vi "Teleop.vi"(10 "Match Info":T1={"Autonomous Elapsed Seconds"=0.0, "TeleOp Elapsed Seconds"=0.0, "Disabled Elapsed Seconds"=0.0, "Visited Autonomous"=FALSE, "Visited TeleOp"=FALSE, "Visited Disabled"=FALSE, "Autonomous Settings"={"Autonomous Style"=enum."Independent", "VI Refnum"=refnum}}, 11 "Call Context":T2) -> ()   [LabVIEW 2020]
doc: "This VI is called for each TeleOp packet received from the DS where the robot is not disabled. It is often used to read from the joysticks and update I/O or to update setpoints for timed control loops. It should complete and return within 20 milliseconds or it may miss DS packets."
uses:
  <vilib>/Rock Robotics/WPI/DriverStation/WPI_DriverStationDerivedRobotMode.ctl
  <vilib>/Rock Robotics/WPI/DriverStation/WPI_DriverStationMatch Info.ctl
  <vilib>/Rock Robotics/WPI/Solenoid/WPI_SolenoidValue.ctl
  <vilib>/Rock Robotics/WPI/Utilities/WPI_GetSetVariantRefNum.vi
  <vilib>/Rock Robotics/WPI/Solenoid/Deprecated/WPI_SolenoidSetBool.vi
  <vilib>/Rock Robotics/Network Tables/NT Write Number.vi
  <vilib>/Rock Robotics/WPI/Solenoid/WPI_SolenoidSetEnum.vi
  Robot Global Data.vi
panel:
  # "April tags"
  # "Retroreflective tape"
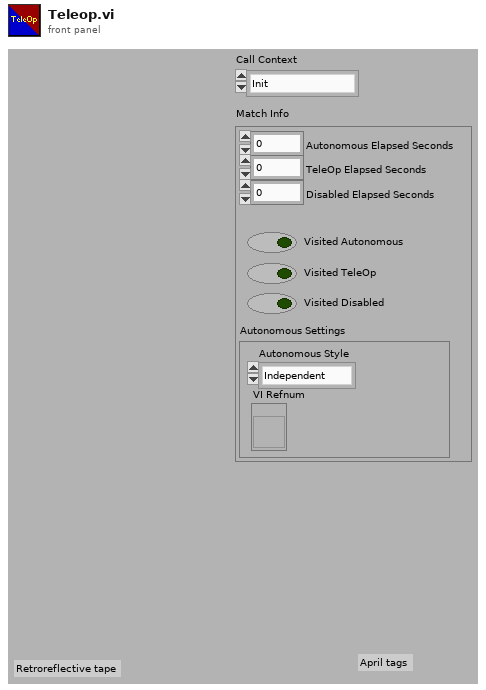
[diagram p1: front panel]
types:
  T1 = typedef "WPI_DriverStationMatch Info.ctl" = cluster{"Autonomous Elapsed Seconds":dbl, "TeleOp Elapsed Seconds":dbl, "Disabled Elapsed Seconds":dbl, "Visited Autonomous":bool, "Visited TeleOp":bool, "Visited Disabled":bool, "Autonomous Settings":cluster{"Autonomous Style":enum16{"Iterative", "Independent"}, "VI Refnum":refnum<vi>}}
  T2 = typedef "WPI_DriverStationDerivedRobotMode.ctl" = enum16{"Init", "Execute", "Stop"}
  T3 = typedef "WPI_SolenoidValue.ctl" = enum16{"Off", "On", "Forward", "Reverse"}
  T4 = typedef "WPI_JoystickDevRef.ctl" = cluster{"Device":T5}
  T5 = typedef "WPI_JoystickDeviceEnum.ctl" = enum16{"USB 0", "USB 1", "USB 2", "USB 3", "USB 4", "USB 5"}
  T6 = cluster{"Axes[0]":dbl, "Axes[1]":dbl, "Axes[2]":dbl, "Axes[3]":dbl, "Axes[4]":dbl, "Axes[5]":dbl, "Axes[6]":dbl, "Axes[7]":dbl, "Axes[8]":dbl}
  T7 = cluster{"Buttons[0]":bool, "Buttons[1]":bool, "Buttons[2]":bool, "Buttons[3]":bool, "Buttons[4]":bool, "Buttons[5]":bool, "Buttons[6]":bool, "Buttons[7]":bool, "Buttons[8]":bool}
  T8 = typedef "WPI_SolenoidDevRef.ctl" = cluster{"DevStatus":errorcluster, "Pneumatics Control Module":u8, "Forward Solenoid Channel":T9, "Reverse Solenoid Channel":T9}
  T9 = typedef "WPI_SolenoidChannel.ctl" = enum8{"Solenoid 0", "Solenoid 1", "Solenoid 2", "Solenoid 3", "Solenoid 4", "Solenoid 5", "Solenoid 6", "Solenoid 7", "Solenoid 8", "Solenoid 9", "Solenoid 10", "Solenoid 11", "Solenoid 12", "Solenoid 13", "Solenoid 14", "Solenoid 15", "Invalid"}
  T10 = typedef "WPI_MotorControlDeviceRef.ctl" = cluster{"DeviceStatus":errorcluster, "Type":T11, "PWM":cluster{"PWM Channel":T12, "DeadBand":T13}, "CAN":cluster{"Device Number":u8, "SetOutput VI Ref":variant, "GetOutput VI Ref":variant, "Enable VI Ref":variant, "Disable VI Ref":variant, "Data":variant}, "Invert":bool, "DIO PWM":cluster{"PWM \"Enable\" Channel":T12, "DIOChannel":T14, "PWM Rate":dbl}}
  T11 = typedef "WPI_MotorControlType.ctl" = enum16{"PWM", "CAN", "DIO PWM"}
  T12 = typedef "FPGA_DIOPWMChannel.ctl" = enum8{"PWM 0", "PWM 1", "PWM 2", "PWM 3", "PWM 4", "PWM 5", "PWM 6", "PWM 7", "PWM 8", "PWM 9", "PWM MXP 0", "PWM MXP 1", "PWM MXP 2", "PWM MXP 3", "PWM MXP 4", "PWM MXP 5", "PWM MXP 6", "PWM MXP 7", "PWM MXP 8", "PWM MXP 9", "Invalid"}
  T13 = typedef "WPI_PWMDeadband.ctl" = cluster{"Name":string, "maxPositivePwm":i32, "minPositivePwm":i32, "centerPwm":i32, "maxNegativePwm":i32, "minNegativePwm":i32, "angularRange":u16}
  T14 = typedef "FPGA_DIOChannel.ctl" = enum8{"DIO 0", "DIO 1", "DIO 2", "DIO 3", "DIO 4", "DIO 5", "DIO 6", "DIO 7", "DIO 8", "DIO 9", "DIO MXP 0", "DIO MXP 1", "DIO MXP 2", "DIO MXP 3", "DIO MXP 4", "DIO MXP 5", "DIO MXP 6", "DIO MXP 7", "DIO MXP 8", "DIO MXP 9", "DIO MXP 10", "DIO MXP 11", "DIO MXP 12", "DIO MXP 13", "DIO MXP 14", "DIO MXP 15", "SPI Port CS1", "SPI Port CS2", "SPI Port CS3", "SPI Port MISO", "SPI Port MOSI", "Invalid"}
  T15 = typedef "WPI_RobotDriveDevRef.ctl" = cluster{"DevStatus":errorcluster, "Motors[]":T10[], "Square Inputs":bool, "Max Output":dbl}
  T16 = cluster{"Motors[][0]":T10, "Motors[][1]":T10, "Motors[][2]":T10, "Motors[][3]":T10, "Motors[][4]":T10, "Motors[][5]":T10, "Motors[][6]":T10, "Motors[][7]":T10, "Motors[][8]":T10}
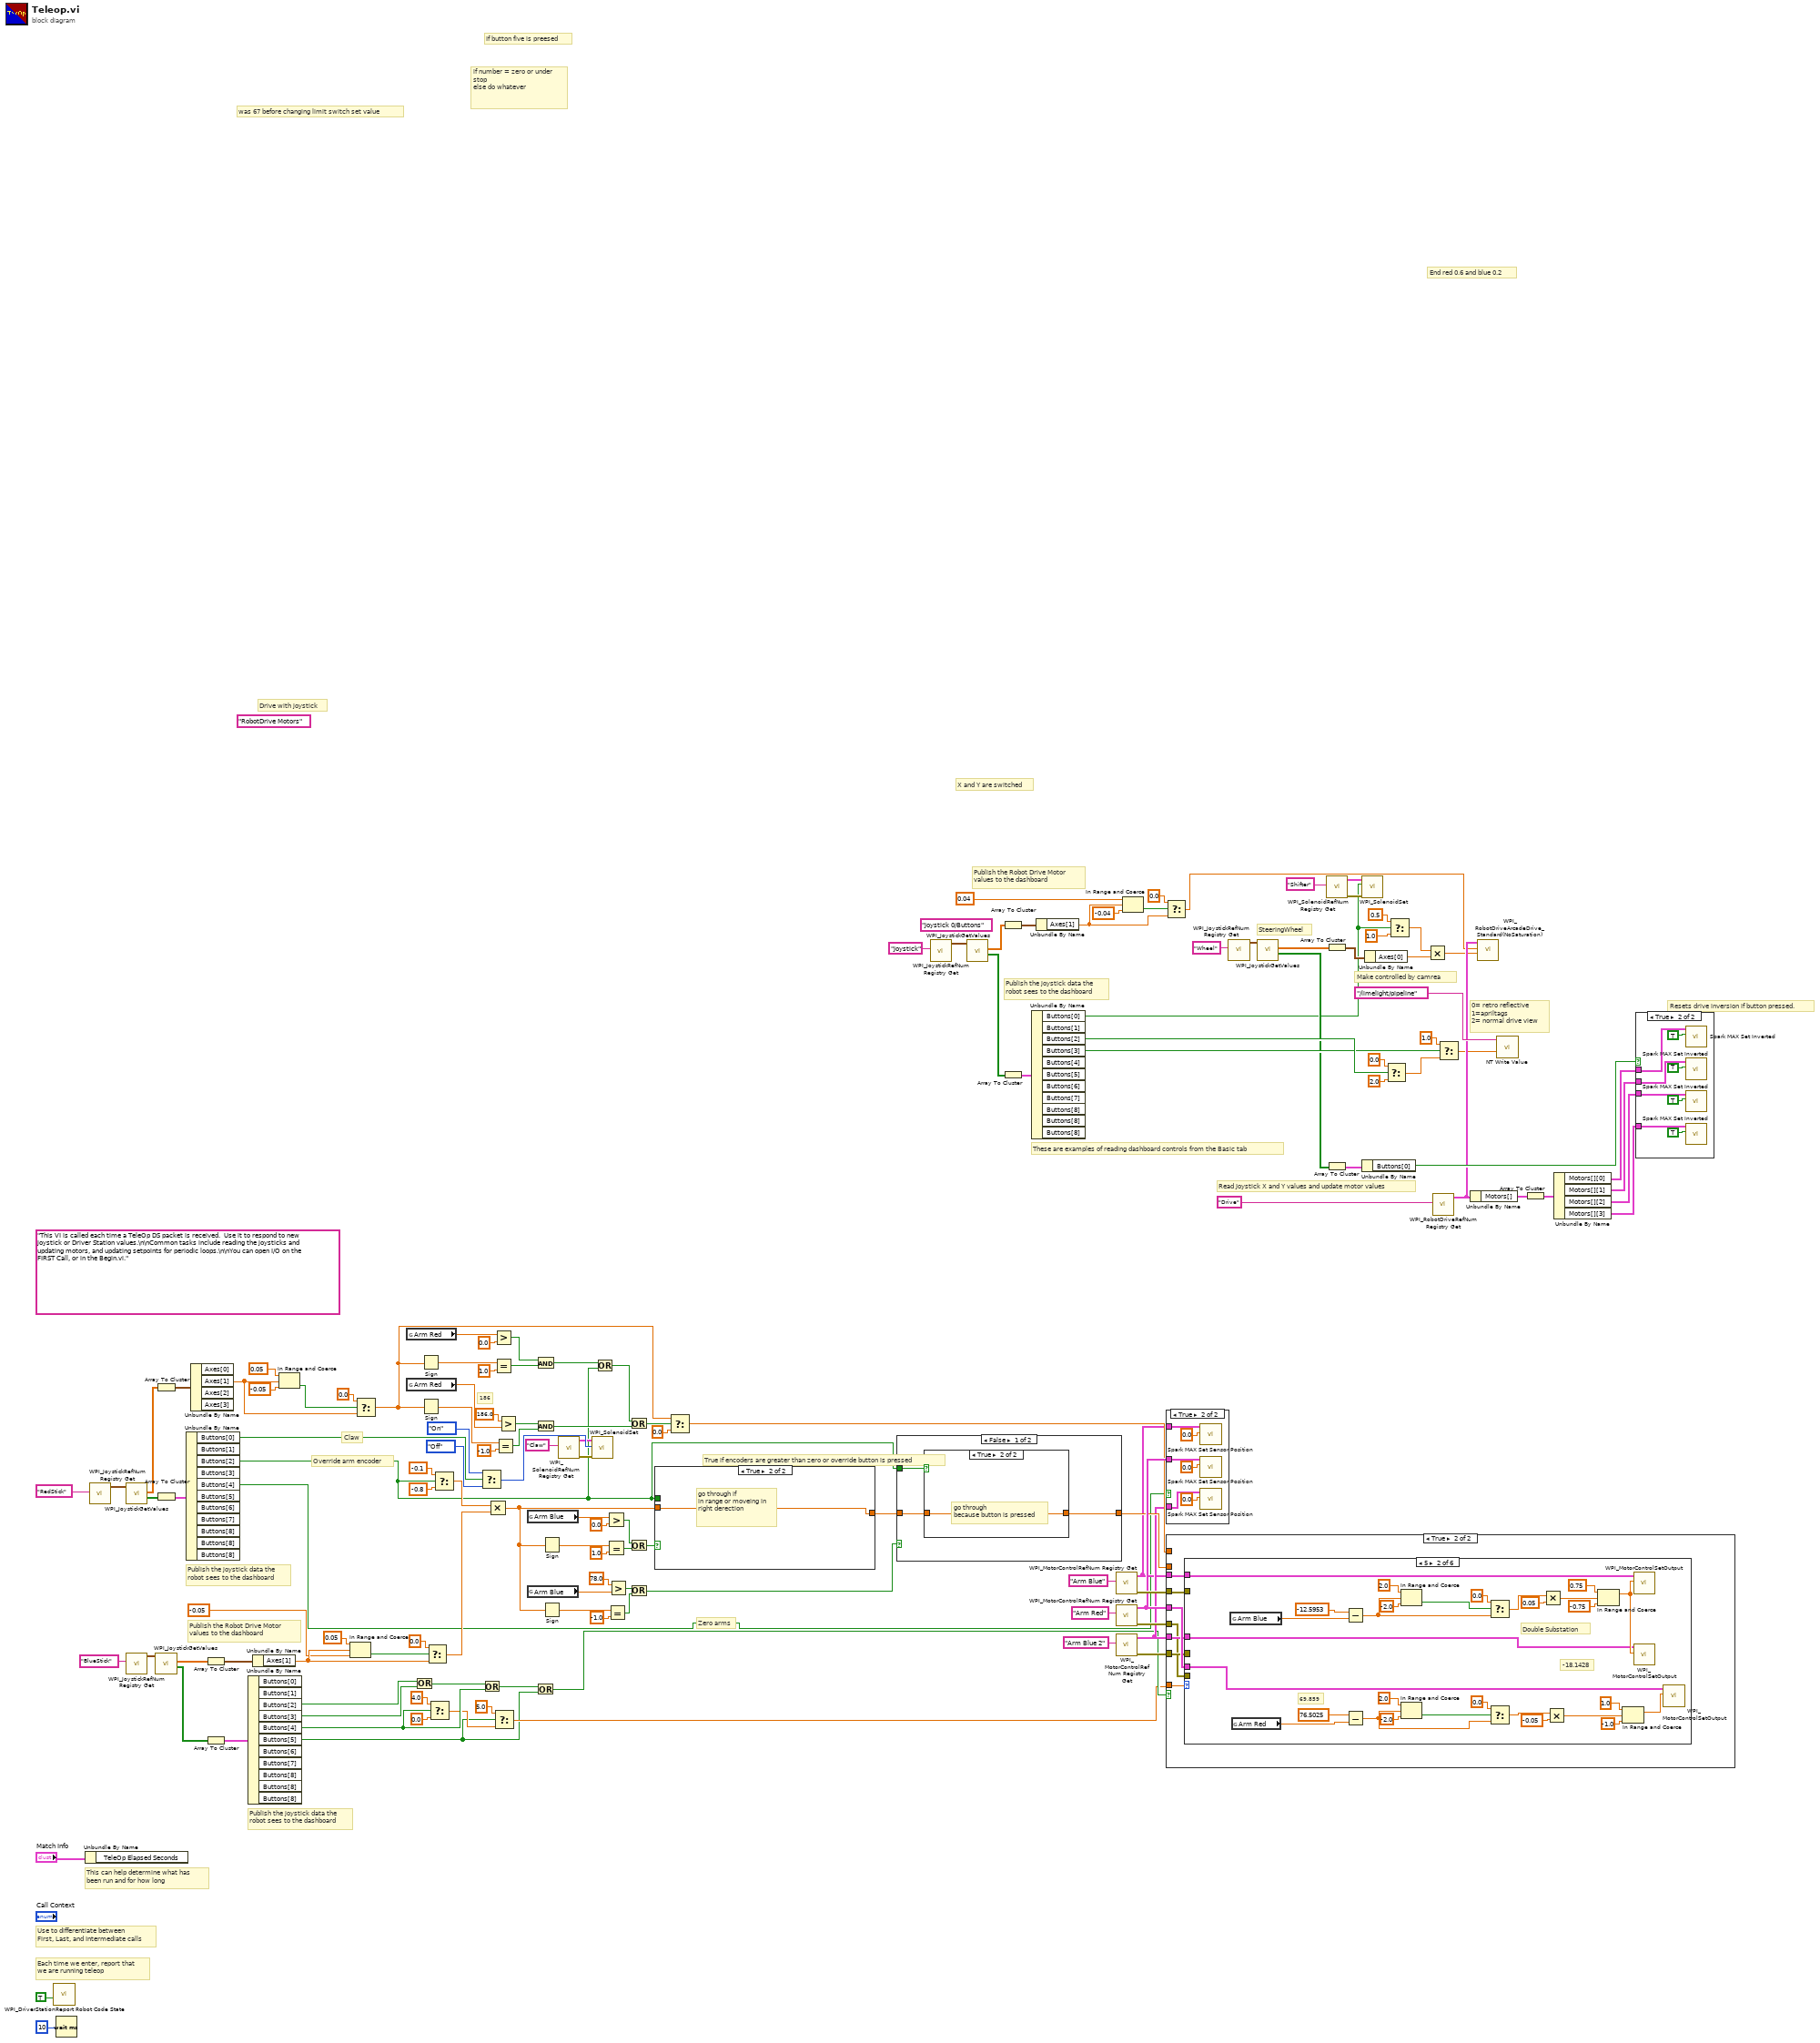
[diagram p0: block diagram]
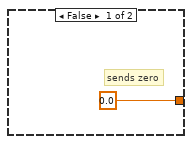
[diagram p2: hidden frame]
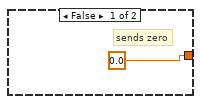
[diagram p5: hidden frame]
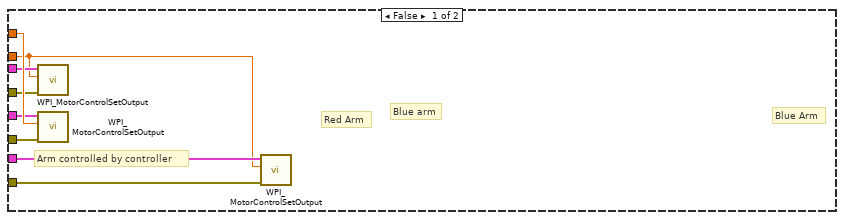
[diagram p8: hidden frame]
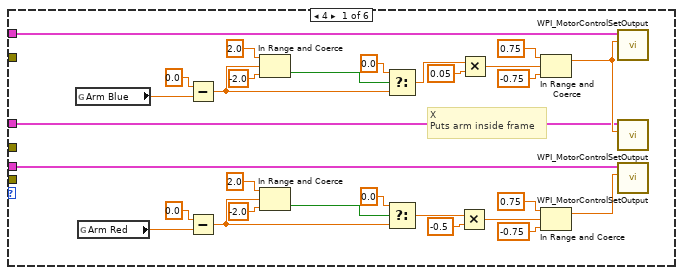
[diagram p9: hidden frame]
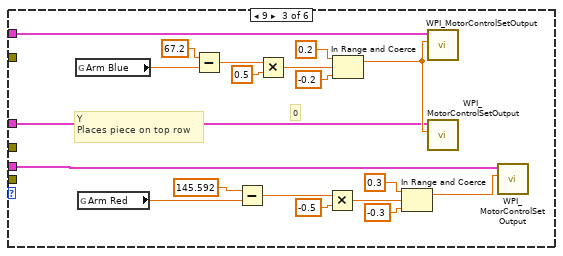
[diagram p10: hidden frame]
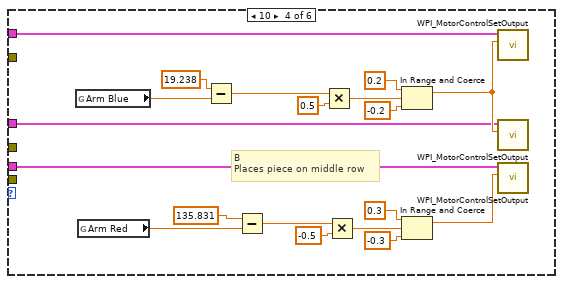
[diagram p11: hidden frame]
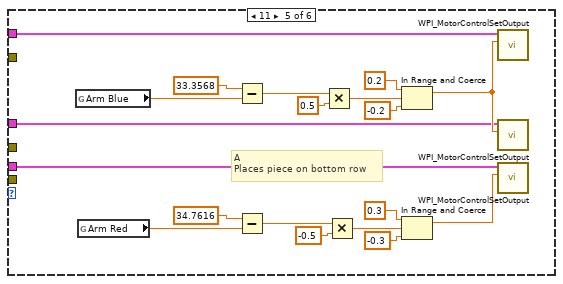
[diagram p12: hidden frame]
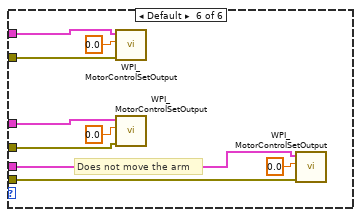
[diagram p13: hidden frame]
diagram:
  (unwired) "RobotDrive Motors" ("Name")
  (unwired) "Joystick 0/Buttons" ("Name")
  (unwired) "This VI is called each time a TeleOp DS packet is received.  Use it to respond to new joystick or Driver Station values.\n\nCommon tasks include reading the joysticks and updating motors, and updating setpoints for periodic loops.\n\nYou can open I/O on the FIRST Call, or in the Begin.vi."
  # "Drive with joystick"
  # "186"
  # "End red 0.6 and blue 0.2"
  # "Zero arms"
  # "Override arm encoder"
  # "Claw"
  # "Publish the Robot Drive Motor\nvalues to the dashboard"
  # "Publish the joystick data the\nrobot sees to the dashboard"
  # "Publish the joystick data the\nrobot sees to the dashboard"
  # "X and Y are switched"
  # "was 67 before changing limit switch set value"
  # "True if encoders are greater than zero or override button is pressed"
  # "if number = zero or under\nstop\nelse do whatever"
  # "If button five is preesed"
  # "Resets drive inversion if button pressed."
  # "0= retro reflective\n1=apriltags\n2= normal drive view"
  # "Make controlled by camrea"
  # "SteeringWheel"
  # "These are examples of reading dashboard controls from the Basic tab"
  # "Publish the Robot Drive Motor\nvalues to the dashboard"
  # "Publish the joystick data the\nrobot sees to the dashboard"
  # "Each time we enter, report that\nwe are running teleop"
  # "Use to differentiate between\nFirst, Last, and Intermediate calls"
  # "This can help determine what has\nbeen run and for how long"
  # "Read Joystick X and Y values and update motor values"
  n1 = call <vilib>:"WPI_DriverStationReport Robot Code State.vi"("TeleOp"=TRUE ("Autonomous")) -> ()  [unwired: 10 in, 1 out]
  n2 = Wait (ms)(milliseconds to wait=u32 10) -> ()  [unwired: 1 out]
  n3 = Unbundle By Name("Match Info") -> ()  [unwired: 1 out]
  n4 = call <vilib>:"WPI_JoystickRefNum Registry Get.vi"("refnum name"="RedStick") -> ("JoystickDevRef"=w39:T4)  [unwired: 1 in, 9 out]
  n5 = call <vilib>:"WPI_JoystickGetValues.vi"("JoystickDevRef"=w39) -> ("Buttons"=w36:bool[], "Axes"=w38:dbl[])  [unwired: 6 in, 3 out]
  n6 = call <vilib>:"WPI_JoystickRefNum Registry Get.vi"("refnum name"="BlueStick") -> ("JoystickDevRef"=w26:T4)  [unwired: 1 in, 9 out]
  n7 = Array To Cluster(array=w38) -> (cluster=w37:T6)
  n8 = Array To Cluster(array=w36) -> (cluster=w35:T7)
  n9 = call <vilib>:"WPI_JoystickGetValues.vi"("JoystickDevRef"=w26) -> ("Buttons"=w29:bool[], "Axes"=w27:dbl[])  [unwired: 6 in, 3 out]
  n10 = Unbundle By Name(w35) -> ("Buttons[0]"=w14:bool, "Buttons[2]"=w22:bool, "Buttons[4]"=w23:bool)  [unwired: 8 out]
  n11 = Unbundle By Name(w37) -> ("Axes[1]"=w18:dbl)  [unwired: 3 out]
  n12 = Array To Cluster(array=w27) -> (cluster=w28:T6)
  n13 = Array To Cluster(array=w29) -> (cluster=w30:T7)
  n14 = Unbundle By Name(w30) -> ("Buttons[2]"=w8:bool, "Buttons[3]"=w9:bool, "Buttons[4]"=w6:bool, "Buttons[5]"=w2:bool)  [unwired: 7 out]
  n15 = Unbundle By Name(w28) -> ("Axes[1]"=w34:dbl)
  n16 = In Range and Coerce(upper limit=0.05, x=w18, lower limit=-0.05) -> (In Range?=w19:bool)  [unwired: 1 out]
  n17 = In Range and Coerce(upper limit=0.05, x=w34, lower limit=-0.05) -> (In Range?=w31:bool)  [unwired: 1 out]
  n18 = Select(t=0.0, s=w19, f=w18) -> (s? t:f=w17:dbl)
  n19 = global read "Robot Global Data.vi" "Arm Red"() -> (w83:dbl)
  n20 = global read "Robot Global Data.vi" "Arm Red"() -> (w77:dbl)
  n21 = Or(x=w8, y=w9) -> (x .or. y?=w13:bool)
  n22 = Sign(1:w17) -> (0:w81:dbl)
  n23 = Sign(1:w17) -> (0:w79:dbl)
  n24 = Select(t=0.0, s=w31, f=w34) -> (s? t:f=w24:dbl)
  n25 = Select(t=4.0, s=w6, f=0.0) -> (s? t:f=w3:dbl)
  n26 = Select(t=-0.1, s=w22, f=-0.8) -> (s? t:f=w45:dbl)
  n27 = Select(t=WPI_SolenoidValue."On" ("Value"), s=w14, f=WPI_SolenoidValue."Off" ("Value")) -> (s? t:f=w62:T3)
  n28 = Or(x=w13, y=w6) -> (x .or. y?=w12:bool)
  n29 = Multiply(x=w45, y=w24) -> (x*y=w42:dbl)
  n30 = Greater?(x=w83, y=0.0) -> (0:w75:bool)
  n31 = Equal?(x=w81, y=1.0) -> (x = y?=w74:bool)
  n32 = Select(t=5.0, s=w2, f=w3) -> (s? t:f=w7:dbl)
  n33 = Equal?(x=w79, y=-1.0) -> (x = y?=w73:bool)
  n34 = Greater?(x=186.0 ("y"), y=w77) -> (0:w72:bool)
  n35 = global read "Robot Global Data.vi" "Arm Blue"() -> (w99:dbl)
  n36 = global read "Robot Global Data.vi" "Arm Blue"() -> (w87:dbl)
  n37 = Or(x=w12, y=w2) -> (x .or. y?=w11:bool)
  n38 = And(x=w75, y=w74) -> (x .and. y?=w71:bool)
  n39 = And(x=w72, y=w73) -> (x .and. y?=w70:bool)
  n40 = Sign(1:w42) -> (0:w96:dbl)
  n41 = Sign(1:w42) -> (0:w91:dbl)
  n42 = call <vilib>:"WPI_SolenoidRefNum Registry Get.vi"("refnum name"="Claw") -> ("error out"=w58:errorcluster, "SolenoidDevRef"=w59:T8)  [unwired: 9 in]
  n43 = call-poly <vilib>:"WPI_SolenoidSet.vi"("error in (no error)"=w58, "Value"=w62, "SolenoidDevRef"=w59) -> ()  [unwired: 7 in, 2 out]
  n44 = Or(x=w71, y=w22) -> (x .or. y?=w69:bool)
  n45 = Greater?(x=w99, y=0.0) -> (0:w98:bool)
  n46 = Equal?(x=w96, y=1.0) -> (x = y?=w94:bool)
  n47 = Equal?(x=w91, y=-1.0) -> (x = y?=w89:bool)
  n48 = Greater?(x=78.0 ("y"), y=w87) -> (0:w92:bool)
  n49 = Or(x=w69, y=w70) -> (x .or. y?=w68:bool)
  n50 = Or(x=w98, y=w94) -> (x .or. y?=w93:bool)
  n51 = Or(x=w92, y=w89) -> (x .or. y?=w88:bool)
  n52 = case shown="True" w93 {
    tunnel: w22 -> [w142 _]
    tunnel: [w141 w145] -> w85
    tunnel: w42 -> [w140 w145]
    frame False {
      n53 = case shown="True" w142 {
        tunnel: [0.0 w144] -> w141
        tunnel: w140 -> [_ w144]
        frame False {
          # "sends zero"
        }
        frame True {
          # "go through\nbecause button is pressed"
        }
      }
    }
    frame True {
      # "go through if\nin range or moveing in right derection"
    }
  }
  n54 = Select(t=w17, s=w68, f=0.0) -> (s? t:f=w66:dbl)
  n55 = case shown="False" w88 {
    tunnel: w22 -> [w148 _]
    tunnel: [w147 w151] -> w84
    tunnel: w85 -> [w146 w151]
    frame False {
      n56 = case shown="True" w148 {
        tunnel: [0.0 w150] -> w147
        tunnel: w146 -> [_ w150]
        frame False {
          # "sends zero"
        }
        frame True {
          # "go through\nbecause button is pressed"
        }
      }
    }
    frame True {
      # "go through if\nin range or moveing in right derection"
    }
  }
  n57 = call <vilib>:"WPI_JoystickRefNum Registry Get.vi"("refnum name"="Joystick") -> ("JoystickDevRef"=w136:T4)  [unwired: 1 in, 9 out]
  n58 = call <vilib>:"WPI_JoystickGetValues.vi"("JoystickDevRef"=w136) -> ("Buttons"=w124:bool[], "Axes"=w134:dbl[])  [unwired: 6 in, 3 out]
  n59 = Array To Cluster(array=w134) -> (cluster=w133:T6)
  n60 = Array To Cluster(array=w124) -> (cluster=w123:T7)
  n61 = Unbundle By Name(w123) -> ("Buttons[0]"=w56:bool, "Buttons[2]"=w115:bool, "Buttons[3]"=w114:bool)  [unwired: 8 out]
  n62 = Unbundle By Name(w133) -> ("Axes[1]"=w47:dbl)
  n63 = call <vilib>:"WPI_MotorControlRefNum Registry Get.vi"("refnum name"="Arm Blue") -> ("error out"=w127:errorcluster, "MotorControlDevRef"=w64:T10)  [unwired: 9 in]
  n64 = call <vilib>:"WPI_MotorControlRefNum Registry Get.vi"("refnum name"="Arm Red") -> ("error out"=w125:errorcluster, "MotorControlDevRef"=w110:T10)  [unwired: 9 in]
  n65 = call <vilib>:"WPI_MotorControlRefNum Registry Get.vi"("refnum name"="Arm Blue 2") -> ("error out"=w111:errorcluster, "MotorControlDevRef"=w65:T10)  [unwired: 9 in]
  n66 = In Range and Coerce(upper limit=0.04, x=w47, lower limit=-0.04) -> (In Range?=w51:bool)  [unwired: 1 out]
  n67 = Select(t=0.0, s=w51, f=w47) -> (s? t:f=w46:dbl)
  n68 = case shown="True" w23 {
    tunnel: w65 -> [_ w157]
    tunnel: w64 -> [_ w156]
    tunnel: w110 -> [_ w155]
    frame False {
    }
    frame True {
      n69 = call <vilib>:"Spark MAX Set Sensor Position.vi"("Position"=0.0, "MotorControlDeviceRef"=w156) -> ()  [unwired: 8 in, 2 out]
      n70 = call <vilib>:"Spark MAX Set Sensor Position.vi"("Position"=0.0, "MotorControlDeviceRef"=w155) -> ()  [unwired: 8 in, 2 out]
      n71 = call <vilib>:"Spark MAX Set Sensor Position.vi"("Position"=0.0, "MotorControlDeviceRef"=w157) -> ()  [unwired: 8 in, 2 out]
    }
  }
  n72 = case shown="True" w11 {
    tunnel: w66 -> [w165 _]
    tunnel: w127 -> [w164 w167]
    tunnel: w64 -> [w163 w170]
    tunnel: w125 -> [w162 w166]
    tunnel: w110 -> [w161 w172]
    tunnel: w65 -> [w160 w171]
    tunnel: w111 -> [w159 w168]
    tunnel: w84 -> [w158 _]
    tunnel: w7 -> [_ w169]
    frame False {
      # "Red Arm"
      # "Blue Arm"
      # "Blue arm"
      # "Arm controlled by controller"
      n73 = call <vilib>:"WPI_MotorControlSetOutput.vi"("error in (no error)"=w164, "Output"=w158, "MotorControlDevRef"=w163) -> ()  [unwired: 6 in, 3 out]
      n74 = call <vilib>:"WPI_MotorControlSetOutput.vi"("error in (no error)"=w162, "Output"=w165, "MotorControlDevRef"=w161) -> ()  [unwired: 6 in, 3 out]
      n75 = call <vilib>:"WPI_MotorControlSetOutput.vi"("error in (no error)"=w159, "Output"=w158, "MotorControlDevRef"=w160) -> ()  [unwired: 6 in, 3 out]
    }
    frame True {
      n76 = case shown="5" w169 {
        tunnel: w172 -> [w185 w202 w231 w250 w271 w292]
        tunnel: w171 -> [w187 w204 w233 w252 w270 w296]
        tunnel: w170 -> [w186 w203 w232 w251 w269 w294]
        tunnel: w168 -> [_ _ _ _ _ w295]
        tunnel: w167 -> [_ _ _ _ _ w293]
        tunnel: w166 -> [_ _ _ _ _ w291]
        frame 4 {
          # "X\nPuts arm inside frame"
          n77 = global read "Robot Global Data.vi" "Arm Blue"() -> (w201:dbl)
          n78 = global read "Robot Global Data.vi" "Arm Red"() -> (w196:dbl)
          n79 = Subtract(x=0.0, y=w201) -> (x-y=w179:dbl)
          n80 = Subtract(x=0.0, y=w196) -> (x-y=w175:dbl)
          n81 = In Range and Coerce(upper limit=2.0, x=w179, lower limit=-2.0) -> (In Range?=w181:bool)  [unwired: 1 out]
          n82 = In Range and Coerce(upper limit=2.0, x=w175, lower limit=-2.0) -> (In Range?=w177:bool)  [unwired: 1 out]
          n83 = Select(t=0.0, s=w181, f=w179) -> (s? t:f=w184:dbl)
          n84 = Select(t=0.0, s=w177, f=w175) -> (s? t:f=w173:dbl)
          n85 = Multiply(x=w173, y=-0.5) -> (x*y=w198:dbl)
          n86 = Multiply(x=w184, y=0.05) -> (x*y=w197:dbl)
          n87 = In Range and Coerce(upper limit=0.75, x=w197, lower limit=-0.75) -> (coerced(x)=w200:dbl)  [unwired: 1 out]
          n88 = In Range and Coerce(upper limit=0.75, x=w198, lower limit=-0.75) -> (coerced(x)=w199:dbl)  [unwired: 1 out]
          n89 = call <vilib>:"WPI_MotorControlSetOutput.vi"("Output"=w200, "MotorControlDevRef"=w186) -> ()  [unwired: 7 in, 3 out]
          n90 = call <vilib>:"WPI_MotorControlSetOutput.vi"("Output"=w200, "MotorControlDevRef"=w187) -> ()  [unwired: 7 in, 3 out]
          n91 = call <vilib>:"WPI_MotorControlSetOutput.vi"("Output"=w199, "MotorControlDevRef"=w185) -> ()  [unwired: 7 in, 3 out]
        }
        frame 5 {
          # "69.859"
          # "-18.1428"
          # "Double Substation"
          n92 = global read "Robot Global Data.vi" "Arm Blue"() -> (w230:dbl)
          n93 = global read "Robot Global Data.vi" "Arm Red"() -> (w225:dbl)
          n94 = Subtract(x=-12.5953, y=w230) -> (x-y=w211:dbl)
          n95 = Subtract(x=76.5025, y=w225) -> (x-y=w207:dbl)
          n96 = In Range and Coerce(upper limit=2.0, x=w211, lower limit=-2.0) -> (In Range?=w213:bool)  [unwired: 1 out]
          n97 = In Range and Coerce(upper limit=2.0, x=w207, lower limit=-2.0) -> (In Range?=w209:bool)  [unwired: 1 out]
          n98 = Select(t=0.0, s=w213, f=w211) -> (s? t:f=w216:dbl)
          n99 = Select(t=0.0, s=w209, f=w207) -> (s? t:f=w205:dbl)
          n100 = Multiply(x=w216, y=0.05) -> (x*y=w226:dbl)
          n101 = Multiply(x=w205, y=-0.05) -> (x*y=w227:dbl)
          n102 = In Range and Coerce(upper limit=0.75, x=w226, lower limit=-0.75) -> (coerced(x)=w229:dbl)  [unwired: 1 out]
          n103 = In Range and Coerce(upper limit=1.0, x=w227, lower limit=-1.0) -> (coerced(x)=w228:dbl)  [unwired: 1 out]
          n104 = call <vilib>:"WPI_MotorControlSetOutput.vi"("Output"=w229, "MotorControlDevRef"=w203) -> ()  [unwired: 7 in, 3 out]
          n105 = call <vilib>:"WPI_MotorControlSetOutput.vi"("Output"=w229, "MotorControlDevRef"=w204) -> ()  [unwired: 7 in, 3 out]
          n106 = call <vilib>:"WPI_MotorControlSetOutput.vi"("Output"=w228, "MotorControlDevRef"=w202) -> ()  [unwired: 7 in, 3 out]
        }
        frame 9 {
          # "0"
          # "Y\nPlaces piece on top row"
          n107 = global read "Robot Global Data.vi" "Arm Blue"() -> (w247:dbl)
          n108 = global read "Robot Global Data.vi" "Arm Red"() -> (w242:dbl)
          n109 = Subtract(x=67.2, y=w247) -> (x-y=w248:dbl)
          n110 = Subtract(x=145.592, y=w242) -> (x-y=w249:dbl)
          n111 = Multiply(x=w248, y=0.5) -> (x*y=w243:dbl)
          n112 = Multiply(x=w249, y=-0.5) -> (x*y=w244:dbl)
          n113 = In Range and Coerce(upper limit=0.2, x=w243, lower limit=-0.2) -> (coerced(x)=w246:dbl)  [unwired: 1 out]
          n114 = In Range and Coerce(upper limit=0.3, x=w244, lower limit=-0.3) -> (coerced(x)=w245:dbl)  [unwired: 1 out]
          n115 = call <vilib>:"WPI_MotorControlSetOutput.vi"("Output"=w246, "MotorControlDevRef"=w232) -> ()  [unwired: 7 in, 3 out]
          n116 = call <vilib>:"WPI_MotorControlSetOutput.vi"("Output"=w246, "MotorControlDevRef"=w233) -> ()  [unwired: 7 in, 3 out]
          n117 = call <vilib>:"WPI_MotorControlSetOutput.vi"("Output"=w245, "MotorControlDevRef"=w231) -> ()  [unwired: 7 in, 3 out]
        }
        frame 10 {
          # "B\nPlaces piece on middle row"
          n118 = global read "Robot Global Data.vi" "Arm Blue"() -> (w266:dbl)
          n119 = global read "Robot Global Data.vi" "Arm Red"() -> (w261:dbl)
          n120 = Subtract(x=19.238, y=w266) -> (x-y=w267:dbl)
          n121 = Subtract(x=135.831, y=w261) -> (x-y=w268:dbl)
          n122 = Multiply(x=w267, y=0.5) -> (x*y=w262:dbl)
          n123 = Multiply(x=w268, y=-0.5) -> (x*y=w263:dbl)
          n124 = In Range and Coerce(upper limit=0.2, x=w262, lower limit=-0.2) -> (coerced(x)=w265:dbl)  [unwired: 1 out]
          n125 = In Range and Coerce(upper limit=0.3, x=w263, lower limit=-0.3) -> (coerced(x)=w264:dbl)  [unwired: 1 out]
          n126 = call <vilib>:"WPI_MotorControlSetOutput.vi"("Output"=w265, "MotorControlDevRef"=w251) -> ()  [unwired: 7 in, 3 out]
          n127 = call <vilib>:"WPI_MotorControlSetOutput.vi"("Output"=w265, "MotorControlDevRef"=w252) -> ()  [unwired: 7 in, 3 out]
          n128 = call <vilib>:"WPI_MotorControlSetOutput.vi"("Output"=w264, "MotorControlDevRef"=w250) -> ()  [unwired: 7 in, 3 out]
        }
        frame 11 {
          # "A\nPlaces piece on bottom row"
          n129 = global read "Robot Global Data.vi" "Arm Blue"() -> (w285:dbl)
          n130 = global read "Robot Global Data.vi" "Arm Red"() -> (w280:dbl)
          n131 = Subtract(x=33.3568, y=w285) -> (x-y=w286:dbl)
          n132 = Subtract(x=34.7616, y=w280) -> (x-y=w287:dbl)
          n133 = Multiply(x=w286, y=0.5) -> (x*y=w281:dbl)
          n134 = Multiply(x=w287, y=-0.5) -> (x*y=w282:dbl)
          n135 = In Range and Coerce(upper limit=0.2, x=w281, lower limit=-0.2) -> (coerced(x)=w284:dbl)  [unwired: 1 out]
          n136 = In Range and Coerce(upper limit=0.3, x=w282, lower limit=-0.3) -> (coerced(x)=w283:dbl)  [unwired: 1 out]
          n137 = call <vilib>:"WPI_MotorControlSetOutput.vi"("Output"=w284, "MotorControlDevRef"=w269) -> ()  [unwired: 7 in, 3 out]
          n138 = call <vilib>:"WPI_MotorControlSetOutput.vi"("Output"=w284, "MotorControlDevRef"=w270) -> ()  [unwired: 7 in, 3 out]
          n139 = call <vilib>:"WPI_MotorControlSetOutput.vi"("Output"=w283, "MotorControlDevRef"=w271) -> ()  [unwired: 7 in, 3 out]
        }
        frame Default {
          # "Does not move the arm"
          n140 = call <vilib>:"WPI_MotorControlSetOutput.vi"("error in (no error)"=w293, "Output"=0.0, "MotorControlDevRef"=w294) -> ()  [unwired: 6 in, 3 out]
          n141 = call <vilib>:"WPI_MotorControlSetOutput.vi"("error in (no error)"=w295, "Output"=0.0, "MotorControlDevRef"=w296) -> ()  [unwired: 6 in, 3 out]
          n142 = call <vilib>:"WPI_MotorControlSetOutput.vi"("error in (no error)"=w291, "Output"=0.0, "MotorControlDevRef"=w292) -> ()  [unwired: 6 in, 3 out]
        }
      }
    }
  }
  n143 = call <vilib>:"WPI_JoystickRefNum Registry Get.vi"("refnum name"="Wheel") -> ("JoystickDevRef"=w131:T4)  [unwired: 9 in, 1 out]
  n144 = call <vilib>:"WPI_JoystickGetValues.vi"("JoystickDevRef"=w131) -> ("Buttons"=w109:bool[], "Axes"=w130:dbl[])  [unwired: 6 in, 3 out]
  n145 = call <vilib>:"WPI_SolenoidRefNum Registry Get.vi"("refnum name"="Shifter") -> ("error out"=w122:errorcluster, "SolenoidDevRef"=w121:T8)  [unwired: 9 in]
  n146 = Array To Cluster(array=w130) -> (cluster=w129:T6)
  n147 = Array To Cluster(array=w109) -> (cluster=w108:T7)
  n148 = call-poly <vilib>:"WPI_SolenoidSet.vi"("error in (no error)"=w122, "Value"=w56, "SolenoidDevRef"=w121) -> ()  [unwired: 7 in, 2 out]
  n149 = Unbundle By Name(w108) -> ("Buttons[0]"=w107:bool)
  n150 = Unbundle By Name(w129) -> ("Axes[0]"=w55:dbl)
  n151 = Select(t=0.0, s=w115, f=2.0) -> (s? t:f=w116:dbl)
  n152 = Select(t=0.5, s=w56, f=1.0) -> (s? t:f=w57:dbl)
  n153 = Multiply(x=w57, y=w55) -> (x*y=w54:dbl)
  n154 = call <vilib>:"WPI_RobotDriveRefNum Registry Get.vi"("refnum name"="Drive") -> ("RobotDriveDevRef"=w104:T15)  [unwired: 1 in, 9 out]
  n155 = Select(t=1.0, s=w114, f=w116) -> (s? t:f=w41:dbl)
  n156 = Unbundle By Name(w104) -> ("Motors[]"=w106:T10[])
  n157 = call <vilib>:"WPI_RobotDriveArcadeDrive_Standard(NoSaturation).vi"("Y axis value"=w54, "X axis value"=w46, "RobotDriveDevRef"=w104) -> ()  [unwired: 1 in, 8 out]
  n158 = call-poly <vilib>:"NT Write Value.vi"("value"=w41, "name"="/limelight/pipeline" ("Name")) -> ()  [unwired: 9 in, 1 out]
  n159 = Array To Cluster(array=w106) -> (cluster=w105:T16)
  n160 = Unbundle By Name(w105) -> ("Motors[][0]"=w103:T10, "Motors[][1]"=w101:T10, "Motors[][2]"=w100:T10, "Motors[][3]"=w102:T10)
  n161 = case shown="True" w107 {
    tunnel: w103 -> [_ w304]
    tunnel: w102 -> [_ w299]
    tunnel: w101 -> [_ w298]
    tunnel: w100 -> [_ w297]
    frame False {
    }
    frame True {
      n162 = call <vilib>:"Spark MAX Set Inverted.vi"("Inverted (F)"=TRUE, "MotorControlDeviceRef in"=w304) -> ()  [unwired: 8 in, 2 out]
      n163 = call <vilib>:"Spark MAX Set Inverted.vi"("Inverted (F)"=TRUE, "MotorControlDeviceRef in"=w298) -> ()  [unwired: 8 in, 2 out]
      n164 = call <vilib>:"Spark MAX Set Inverted.vi"("Inverted (F)"=TRUE, "MotorControlDeviceRef in"=w297) -> ()  [unwired: 8 in, 2 out]
      n165 = call <vilib>:"Spark MAX Set Inverted.vi"("Inverted (F)"=TRUE, "MotorControlDeviceRef in"=w299) -> ()  [unwired: 8 in, 2 out]
    }
  }
